vi "Read Variable_Values.vi"(8 "error in (no error)":errorcluster, 11 "muExpr in":refnum<class "mupExpr.lvclass">) -> (0 "error out":errorcluster, 2 "varValues":dbl[](array[numeric]), 3 "muExpr out":refnum<class "mupExpr.lvclass">)   [LabVIEW 2015, in "mupExpr.lvclass"]
uses:
  mupExpr.lvclass
  mupExpr.lvclass/mupExpr.ctl
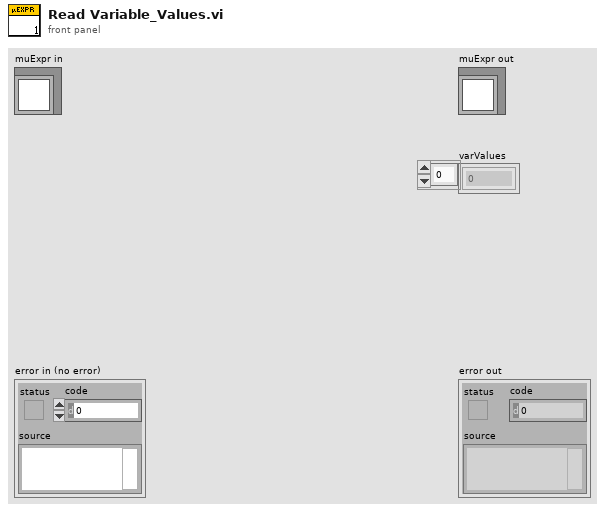
[diagram p1: front panel]
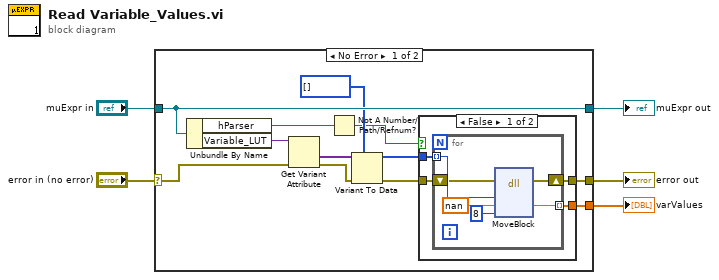
[diagram p0: block diagram]
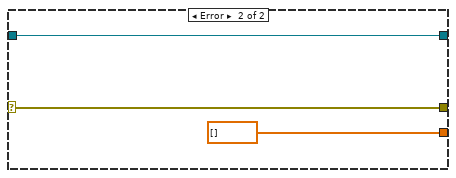
[diagram p3: hidden frame]
diagram:
  n1 = case shown="No Error" "error in (no error)" {
    selector: "error in (no error)" -> [w10 w31]
    tunnel: [w9 w31] -> w4
    tunnel: [w17 w30] -> w2
    tunnel: "muExpr in" -> [w17 w30]
    tunnel: [w8 dbl[] [] ("pd")] -> w1
    frame No Error {
      n2 = Unbundle By Name(w17) -> ("hParser"=w7:refnum<data-value>, "Variable_LUT"=w16:variant)
      n3 = Get Variant Attribute(Variant=w16, error in=w10) -> (values=w15:variant[], error out=w13:errorcluster)  [unwired: 2 in, 2 out]
      n4 = Not A Number/Path/Refnum?(number/path/refnum=w7) -> (NaN/Path/Refnum?=w6:bool)
      n5 = Variant To Data(error in=w13, type=u64[] [], Variant=w15) -> (data=w12:u64[], error out=w11:errorcluster)
      n6 = case shown="False" w6 {
        tunnel: w12 -> [w21 _]
        tunnel: w11 -> [w20 w28]
        tunnel: [w19 w28] -> w9
        tunnel: [w18 _] -> w8
        frame False {
          n7 = for {
            tunnel: w21 -> [w26] mode=indexing
            tunnel: [w23] -> w18 mode=indexing
            shift-right: [w22] -> w19
            shift-left: w20 -> [w25]
            n8 = dll-call lib="LabVIEW" fn="MoveBlock"(error in=w25, "ps"=w26, "pd"=nan, "size"=8) -> (error out=w22:errorcluster, "pd"=w23:dbl)  [unwired: 5 in, 1 out]
          }
        }
        frame True {
        }
      }
    }
    frame Error {
    }
  }
  "error out" <- w4
  "muExpr out" <- w2
  "varValues" <- w1
